vi "Run All Tests.vi"() -> (0 "error out":errorcluster)   [LabVIEW 2013]
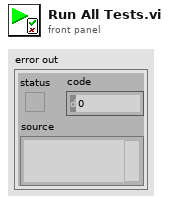
[diagram p1: front panel]
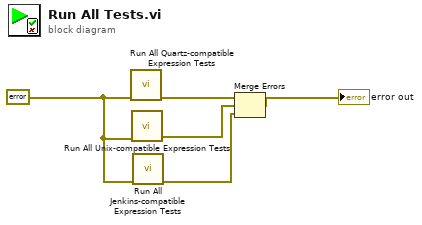
[diagram p0: block diagram]
diagram:
  w2 = errorcluster {"status"=FALSE, "code"=0, "source"=""} ("error in")
  n1 = call "Run All Quartz-compatible Expression Tests.vi"("error in"=w2) -> ("error out"=w5:errorcluster)  [unwired: 10 in]
  n2 = call "Run All Unix-compatible Expression Tests.vi"("error in"=w2) -> ("error out"=w3:errorcluster)  [unwired: 10 in]
  n3 = call "Run All Jenkins-compatible Expression Tests.vi"("error in"=w2) -> ("error out"=w1:errorcluster)  [unwired: 10 in]
  n4 = Merge Errors(w5, w3, w1) -> (→"error out":errorcluster)
